vi "Alarm_Logic.vi"(0 "Measurement_Data":T1, 5 "Temperature_Limit":dbl=30.0, 7 "Humidity_Limit":dbl=65.0, 9 "Previous_Temperature_Alarm":bool, 11 "Previous_Humidity_Alarm":bool, 12 "Previous_Water_Alarm":bool) -> (2 "Send_Notification":bool, 4 "Temperature_Alarm":bool, 6 "Humidity_Alarm":bool, 8 "Water_Alarm":bool, 10 "New_Temperature_Alarm":bool, 14 "New_Water_Alarm":bool, 15 "New_Humidity_Alarm":bool)   [LabVIEW 2026]
uses:
  Measurement_Data.ctl
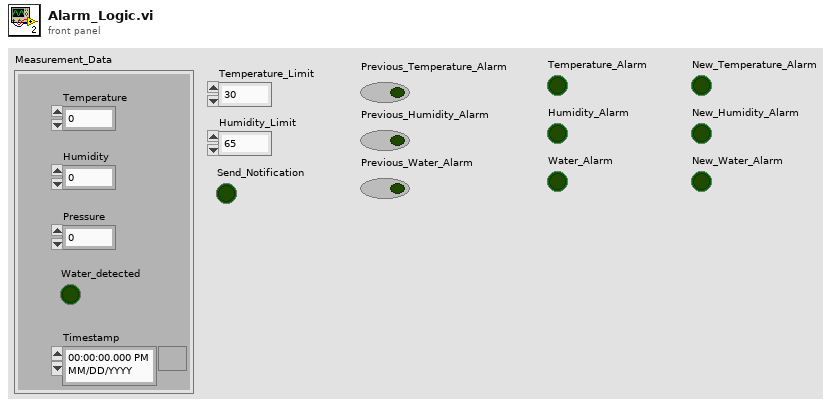
[diagram p1: front panel]
types:
  T1 = typedef "Measurement_Data.ctl" = cluster{"Temperature":dbl, "Humidity":dbl, "Pressure":dbl, "Water_detected":bool, "Timestamp":timestamp}
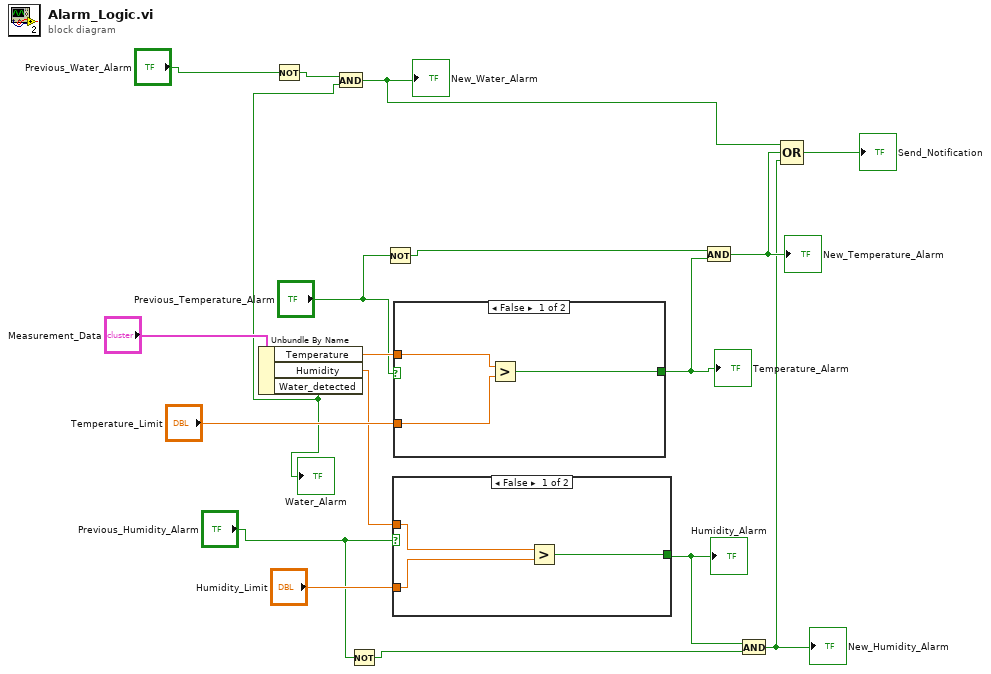
[diagram p0: block diagram]
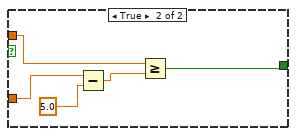
[diagram p2: hidden frame]
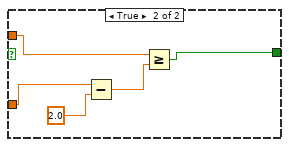
[diagram p3: hidden frame]
diagram:
  n1 = Unbundle By Name("Measurement_Data") -> ("Temperature"=w17:dbl, "Humidity"=w15:dbl, "Water_detected"=w5:bool)
  "Water_Alarm" <- w5
  n2 = Not(x="Previous_Water_Alarm") -> (.not. x?=w6:bool)
  n3 = And(x=w6, y=w5) -> (x .and. y?=w4:bool)
  "New_Water_Alarm" <- w4
  n4 = Not(x="Previous_Humidity_Alarm") -> (.not. x?=w8:bool)
  n5 = Not(x="Previous_Temperature_Alarm") -> (.not. x?=w11:bool)
  n6 = case shown="False" "Previous_Humidity_Alarm" {
    tunnel: w15 -> [w21 w23]
    tunnel: "Humidity_Limit" -> [w20 w24]
    tunnel: [w19 w22] -> w10
    frame False {
      n7 = Greater?(x=w21, y=w20) -> (0:w19:bool)
    }
    frame True {
      n8 = Subtract(x=w24, y=5.0) -> (x-y=w25:dbl)
      n9 = Greater Or Equal?(x=w23, y=w25) -> (x >= y?=w22:bool)
    }
  }
  "Humidity_Alarm" <- w10
  n10 = case shown="False" "Previous_Temperature_Alarm" {
    tunnel: w17 -> [w29 w32]
    tunnel: "Temperature_Limit" -> [w28 w34]
    tunnel: [w27 w30] -> w13
    frame False {
      n11 = Greater?(x=w29, y=w28) -> (0:w27:bool)
    }
    frame True {
      n12 = Subtract(x=w34, y=2.0) -> (x-y=w31:dbl)
      n13 = Greater Or Equal?(x=w32, y=w31) -> (x >= y?=w30:bool)
    }
  }
  "Temperature_Alarm" <- w13
  n14 = And(x=w11, y=w13) -> (x .and. y?=w3:bool)
  "New_Temperature_Alarm" <- w3
  n15 = And(x=w10, y=w8) -> (x .and. y?=w2:bool)
  "New_Humidity_Alarm" <- w2
  n16 = Compound Arithmetic op=OR(w4, w3, w2) -> (→"Send_Notification":bool)
